vi "Edit Line.vi"(8 "error in":errorcluster, 10 "Line Name":string, 11 "References":T1) -> (0 "error out":errorcluster, 2 "change?":bool)   [LabVIEW 2015, in "J1939 editor node.lvclass"]
doc: "This VI edits the properties of a line. It will unlink channels and tags and create new links to channels and tags."
uses:
  J1939 editor node.lvclass
  <vilib>/NI/DCAF/Tag Editor Core/Table API/Table Manager/object ref.ctl
  <vilib>/NI/DCAF/Tag Editor Core/Configuration Editor/Classes/Engine Parent/Engine Parent Editor Node.lvclass
  <vilib>/NI/DCAF/Tag Editor Core/Configuration Editor/Classes/Module editor node/module editor node.lvclass
  module/configuration/J1939 configuration.lvclass
  module/configuration/J1939 configuration.lvclass/J1939 configuration.ctl
  <vilib>/NI/Configuration Framework/serializable configuration/NISE_CEF_serializable configuration.lvclass/NISE_CEF_serializable configuration.ctl
  <vilib>/Utility/LVClass/Get LV Class Name.vi
  <vilib>/NI/Configuration Framework/error generator/NISE_error generator.vi
  <vilib>/NI/Tag Bus Module Framework/channel/TBM channel.lvclass
  <vilib>/NI/Configuration Framework/serializable configuration/NISE_CEF_serializable configuration.lvclass
  <vilib>/NI/DCAF/Tag Editor Core/Table API/Table Manager/Table Manager.lvclass
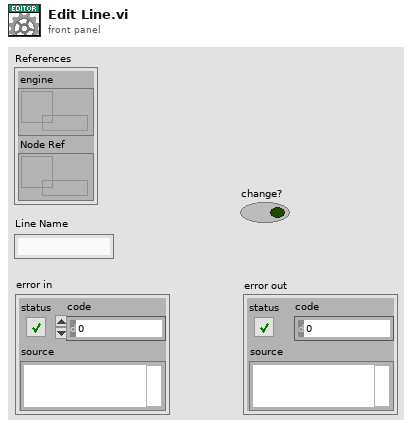
[diagram p1: front panel]
types:
  T1 = typedef "Table Manager.lvlib/Table Manager.lvclass/object ref.ctl" = cluster{"engine":refnum<data-value>, "Node Ref":refnum<data-value>}
  T2 = typedef "J1939 configuration.lvclass/Line.ctl" = cluster{"channel":refnum<class "TBM channel.lvclass">, "XNET Signal":refnum<k21>}
  T3 = typedef "J1939 editor node.lvclass/Mappings.ctl" = cluster{"Line":T2, "Maps":T4[]}
  T4 = typedef "J1939 editor node.lvclass/Map.ctl" = cluster{"channel":refnum<class "TBM channel.lvclass">, "tag name":string}
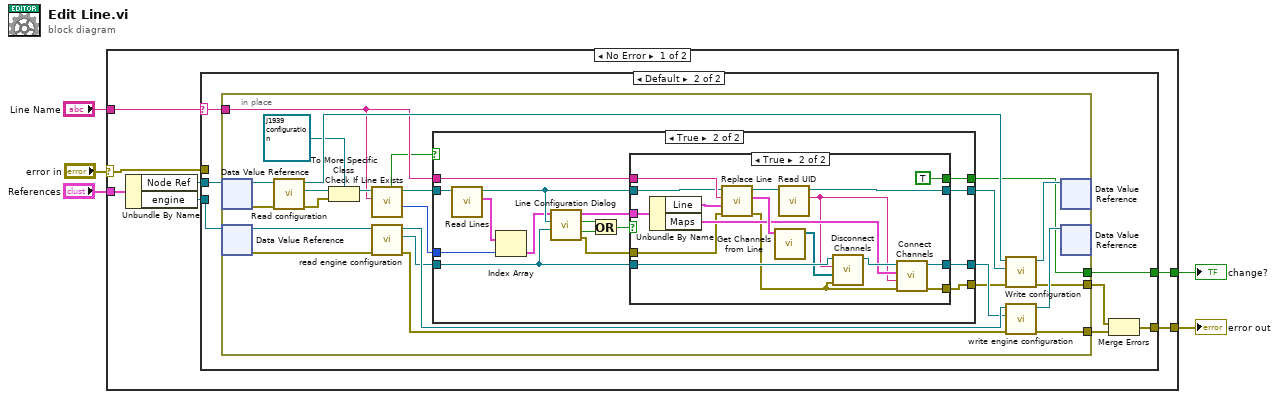
[diagram p0: block diagram]
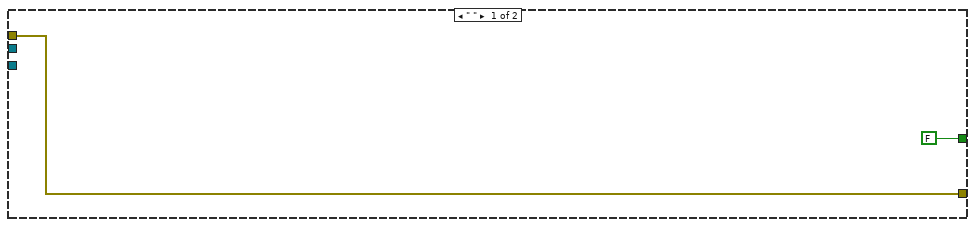
[diagram p2: hidden frame]
diagram:
  n1 = case shown="No Error" "error in" {
    selector: "error in" -> [w6 w83]
    tunnel: "References" -> [w10 _]
    tunnel: "Line Name" -> [w7 _]
    tunnel: [w9 w83] -> w2
    tunnel: [w8 _] -> w1
    frame No Error {
      n2 = Unbundle By Name(w10) -> ("Node Ref"=w12:refnum<data-value>, "engine"=w11:refnum<data-value>)
      n3 = case shown="Default" w7 {
        selector: w7 -> [_ w15]
        tunnel: w12 -> [_ w21]
        tunnel: w11 -> [_ w20]
        tunnel: [w13 w17] -> w9
        tunnel: [FALSE ("change?") w16] -> w8
        tunnel: w6 -> [w13 _]
        frame " " {
        }
        frame Default {
          n4 = in-place {
            in-place-border: [w26] -> w19
            in-place-border: [w42] -> w18
            in-place-border: [w25] -> w16
            in-place-border: w15 -> [w31]
            n5 = in-place-dvr #1(w21) -> (w38:refnum<class "module editor node.lvclass">, w32:errorcluster)
            n6 = in-place-dvr #2(w20) -> (w45:refnum<class "Engine Parent Editor Node.lvclass">, w44:errorcluster)
            n7 = call-dynamic "Read configuration.vi"("error in"=w32, "NISE_CEF_serializable node in"=w38) -> ("error out"=w35:errorcluster, "configuration"=w36:refnum<class "NISE_CEF_serializable configuration.lvclass">, "NISE_CEF_serializable node out"=w37:refnum<class "module editor node.lvclass">)  [unwired: 7 in]
            n8 = To More Specific Class(target class=refnum<class "J1939 configuration.lvclass"> refnum ("tag bus configurable plugin module configuration"), reference=w36, error in=w35) -> (specific class reference=w33:refnum<class "J1939 configuration.lvclass">)  [unwired: 1 out]
            n9 = call-dynamic "Check If Line Exists.vi"("Name to Locate"=w31, "J1939 configuration in"=w33) -> ("Index"=w28:i32, "J1939 configuration out"=w29:refnum<class "J1939 configuration.lvclass">, "Found?"=w23:bool)  [unwired: 5 in, 2 out]
            n10 = call <vilib>:"read engine configuration.vi"("error in"=w44, "Engine Parent Editor Node in"=w45) -> ("error out"=w40:errorcluster, "engine configuration"=w27:refnum<class "engine configuration.lvclass">, "Engine Parent Editor Node out"=w41:refnum<class "Engine Parent Editor Node.lvclass">)  [unwired: 7 in]
            n11 = case shown="True" w23 {
              tunnel: w29 -> [w47 w61]
              tunnel: w27 -> [w46 w52]
              tunnel: w31 -> [_ w63]
              tunnel: [w47 w55] -> w30
              tunnel: w28 -> [_ w58]
              tunnel: [_ w54] -> w25
              tunnel: [w46 w53] -> w24
              tunnel: [_ w48] -> w22
              frame False {
              }
              frame True {
                n12 = call "Read Lines.vi"("J1939 configuration in"=w61) -> ("Lines"=w59:T2[], "J1939 configuration out"=w60:refnum<class "J1939 configuration.lvclass">)  [unwired: 8 in, 1 out]
                n13 = Index Array(array=w59, index=w58) -> (element=w57:T2)
                n14 = call "Line Configuration Dialog.vi"("engine configuration in"=w52, "tag bus configurable plugin module configuration"=w60, "Line"=w57) -> ("error out"=w62:errorcluster, "success"=w50:bool, "changed"=w49:bool, "Mappings out"=w56:T3)  [unwired: 5 in]
                n15 = Or(x=w49, y=w50) -> (x .or. y?=w51:bool)
                n16 = case shown="True" w51 {
                  tunnel: w63 -> [_ w82]
                  tunnel: w52 -> [w64 w81]
                  tunnel: w62 -> [_ w67]
                  tunnel: w60 -> [w65 w77]
                  tunnel: w56 -> [_ w76]
                  tunnel: [w65 w74] -> w55
                  tunnel: [_ TRUE ("change?")] -> w54
                  tunnel: [w64 w69] -> w53
                  tunnel: [_ w68] -> w48
                  frame False {
                  }
                  frame True {
                    n17 = Unbundle By Name(w76) -> ("Line"=w75:T2, "Maps"=w72:T4[])
                    n18 = call "Replace Line.vi"("error in"=w67, "New Line"=w75, "Line Name"=w82, "J1939 configuration in"=w77) -> ("error out"=w66:errorcluster, "Old Line"=w79:T2, "J1939 configuration out"=w80:refnum<class "J1939 configuration.lvclass">)  [unwired: 5 in]
                    n19 = call "Get Channels from Line.vi"("Line"=w79) -> ("Channels"=w78:refnum<class "TBM channel.lvclass">[])  [unwired: 10 in]
                    n20 = call <vilib>:"Read UID.vi"("configuration in"=w80) -> ("instance id"=w71:string, "configuration out"=w74:refnum<class "J1939 configuration.lvclass">)  [unwired: 8 in, 1 out]
                    n21 = call "Disconnect Channels.vi"("error in (no error)"=w66, "Deleted Channels"=w78, "instance id"=w71, "Engine Configuration in"=w81) -> ("Engine Configuration out"=w73:refnum<class "engine configuration.lvclass">)  [unwired: 6 in, 1 out]
                    n22 = call "Connect Channels.vi"("error in (no error)"=w66, "instance id"=w71, "Maps"=w72, "Engine Configuration in"=w73) -> ("error out"=w68:errorcluster, "Engine Configuration out"=w69:refnum<class "engine configuration.lvclass">)  [unwired: 6 in]
                  }
                }
              }
            }
            n23 = call-dynamic "Write configuration.vi"("error in"=w22, "configuration"=w30, "NISE_CEF_serializable node in"=w37) -> ("error out"=w26:errorcluster, "NISE_CEF_serializable node out"=w39:refnum<class "module editor node.lvclass">)  [unwired: 7 in]
            n24 = call <vilib>:"write engine configuration.vi"("error in"=w40, "engine configuration"=w24, "Engine Parent Editor Node in"=w41) -> ("error out"=w42:errorcluster, "Engine Parent Editor Node out"=w43:refnum<class "Engine Parent Editor Node.lvclass">)  [unwired: 7 in]
            n25 = in-place-dvr #1(w39) -> ()  [unwired: 2 out]
            n26 = in-place-dvr #2(w43) -> ()  [unwired: 2 out]
          }
          n27 = Merge Errors(w19, w18) -> (w17:errorcluster)
        }
      }
    }
    frame Error {
    }
  }
  "change?" <- w1
  "error out" <- w2
